vi "Copy .LLB to NI VeriStand dir.vi"(5 "Files Generated by Build":path[](array[path]), 6 "Top Level/Always Included VIs":path[](array[path]), 7 "Destination Path":path, 8 "error in (no error)":errorcluster, 9 "Target Name":string, 10 "Build Specification Name":string, 11 "Project Path":path) -> (0 "error out":errorcluster)   [LabVIEW 2024]
doc: "This VI is called after each run of a build specification. The VI will copy the generated LLB (Engine or System Explorer) into the VeriStand Custom Device folder (...\\Documents\\National Instruments\\NI VeriStand 2013...)."
uses:
  <vilib>/Utility/sysdir.llb/System Directory Type.ctl
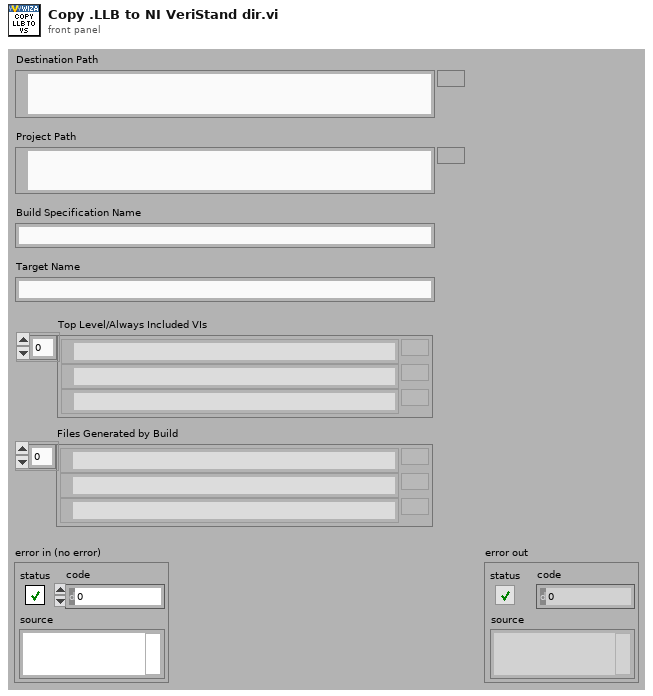
[diagram p1: front panel]
types:
  T1 = typedef "System Directory Type.ctl" = i32
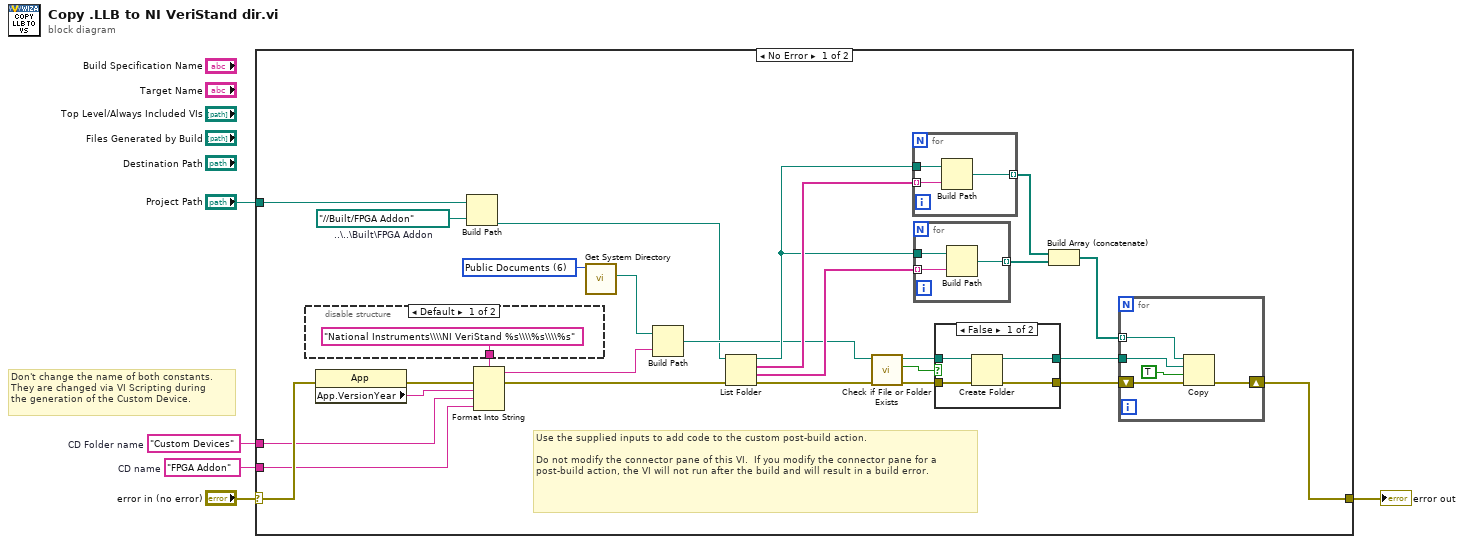
[diagram p0: block diagram]
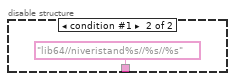
[diagram p2: hidden frame]
diagram:
  w1 = "FPGA Addon"  # CD name
  w2 = "Custom Devices"  # CD Folder name
  # "Don't change the name of both constants.\nThey are changed via VI Scripting during\nthe generation of the Custom Device."
  n1 = case shown="No Error" "error in (no error)" {
    selector: "error in (no error)" -> [w15 w52]
    tunnel: [w17 w52] -> w3
    tunnel: "Project Path" -> [w13 _]
    tunnel: w2 -> [w9 _]
    tunnel: w1 -> [w7 _]
    frame No Error {
      w6 = path "../../Built/FPGA Addon"  # ..\..\Built\FPGA Addon
      w20 = T1 6 items=["User Home"=0, "User Desktop"=1, "User Documents"=2, "User Application Data"=3, "User Preferences"=4, "User Temporary"=5, "Public Documents"=6, "Public Application Data"=7, "Public Preferences"=8, "Public Cache"=13, "System Core Libraries"=9, "System Installed Libraries"=10, "Application Files"=11, "Boot Volume Root"=12] ("system directory type")
      # "Use the supplied inputs to add code to the custom post-build action.\n\nDo not modify the connector pane of this VI.  If you modify the connector pane for a post-build action, the VI will not run after the build and will result in a build error."
      n2 = disable-structure shown="Default" {
        disable-tunnel: ["National Instruments\\\\NI VeriStand %s\\\\%s\\\\%s" ("name or relative path") "lib64//niveristand%s//%s//%s" ("name or relative path")] -> w8
        frame condition #0 (active) {
        }
        frame condition #1 {
        }
      }
      n3 = property class="App"(error in=w15) -> (error out=w19:errorcluster, "App.VersionYear"=w18:string)  [unwired: 1 in, 1 out]
      n4 = Build Path(base path=w13, name or relative path=w6) -> (appended path=w10:path)
      n5 = Format Into String(format string=w8, error in=w19, w18, w9, w7) -> (resulting string=w22:string, error out=w14:errorcluster)  [unwired: 1 in]
      n6 = call <vilib>:"Get System Directory.vi"("system directory type"=w20) -> ("system directory"=w21:path)  [unwired: 10 in]
      n7 = Build Path(base path=w21, name or relative path=w22) -> (appended path=w16:path)
      n8 = List Folder(path=w10, error in=w14) -> (path out=w25:path, filenames=w32:string[], folder names=w26:string[], error out=w23:errorcluster)  [unwired: 2 in]
      n9 = call <vilib>:"Check if File or Folder Exists.vi"("error in (no error)"=w23, "path"=w16) -> ("error out"=w27:errorcluster, "file or folder exists?"=w29:bool, "dup path"=w28:path)  [unwired: 7 in]
      n10 = for {
        tunnel: w32 -> [w50] mode=indexing
        tunnel: w25 -> [w51]
        tunnel: [w49] -> w31 mode=indexing
        n11 = Build Path(base path=w51, name or relative path=w50) -> (appended path=w49:path)
      }
      n12 = for {
        tunnel: w26 -> [w47] mode=indexing
        tunnel: w25 -> [w48]
        tunnel: [w46] -> w24 mode=indexing
        n13 = Build Path(base path=w48, name or relative path=w47) -> (appended path=w46:path)
      }
      n14 = case shown="False" w29 {
        tunnel: w28 -> [w38 w40]
        tunnel: w27 -> [w37 w39]
        tunnel: [w36 w40] -> w12
        tunnel: [w35 w39] -> w11
        frame False {
          n15 = Create Folder(path (use dialog)=w38, error in=w37) -> (created path=w36:path, error out=w35:errorcluster)  [unwired: 1 in, 1 out]
        }
        frame True {
        }
      }
      n16 = Build Array (concatenate)(w31, w24) -> (w30:path[])
      n17 = for {
        tunnel: w30 -> [w42] mode=indexing
        shift-right: [w43] -> w17
        shift-left: w11 -> [w44]
        tunnel: w12 -> [w41]
        n18 = Copy(8:w44, 9:TRUE ("overwrite (F)"), 10:w41, 11:w42) -> (0:w43:errorcluster)  [unwired: 1 in, 2 out]
      }
    }
    frame Error {
    }
  }
  "error out" <- w3
